vi "FT10xx系列_T1_sample_1.0.3.vi"() -> ()   [LabVIEW 2017]
uses:
  National Instruments/LabVIEW 2017/user.lib/smncsftmt/smncsftmt.lvlib
panel:
  out "数值 2":i32
  in  "分辨率":T1(ring)
  in  "分辨":T2(ring)
  in  "停止按钮":bool
  out "START 计数率":u32
  in  "开始测试":bool
  out "CH8 计数率":u32
  out "CH7 计数率":u32
  out "CH6 计数率":u32
  out "CH5 计数率":u32
  out "CH4 计数率":u32
  out "CH3 计数率":u32
  out "CH2 计数率":u32
  out "CH1 计数率":u32
  in  "Delay 8":dbl min=-1000.0 max=1000.0 step=0.1 format="%.1fns"
  in  "Delay 7":dbl min=-1000.0 max=1000.0 step=0.1 format="%.1fns"
  in  "Delay 6":dbl min=-1000.0 max=1000.0 step=0.1 format="%.1fns"
  in  "Delay 5":dbl min=-1000.0 max=1000.0 step=0.1 format="%.1fns"
  in  "Delay 4":dbl min=-1000.0 max=1000.0 step=0.1 format="%.1fns"
  in  "Delay 3":dbl min=-1000.0 max=1000.0 step=0.1 format="%.1fns"
  in  "Delay2":dbl min=-1000.0 max=1000.0 step=0.1 format="%.1fns"
  in  "Delay":dbl min=-1000.0 max=1000.0 step=0.1 format="%.1fns"
  in  "单选按钮 2":T3(radio)
  in  "保存路径":path=path "D:/siminics"
  in  "最大计数":u64=65535 min=1 max=4294967295 step=1
  in  "总采集时长（s)":sgl=1.0 min=0.1 max=604080 step=0.1
  out "TDC Controller":u64[](graph)
  out "采集次数":u32
  out "峰值计数":u32
  out "error out":errorcluster caption="错误输出"
  out "峰值时间点(ps)":u32
  out "已连接？":bool
  # "FT10XX系列直方图(T1)"
  # "通道选择"
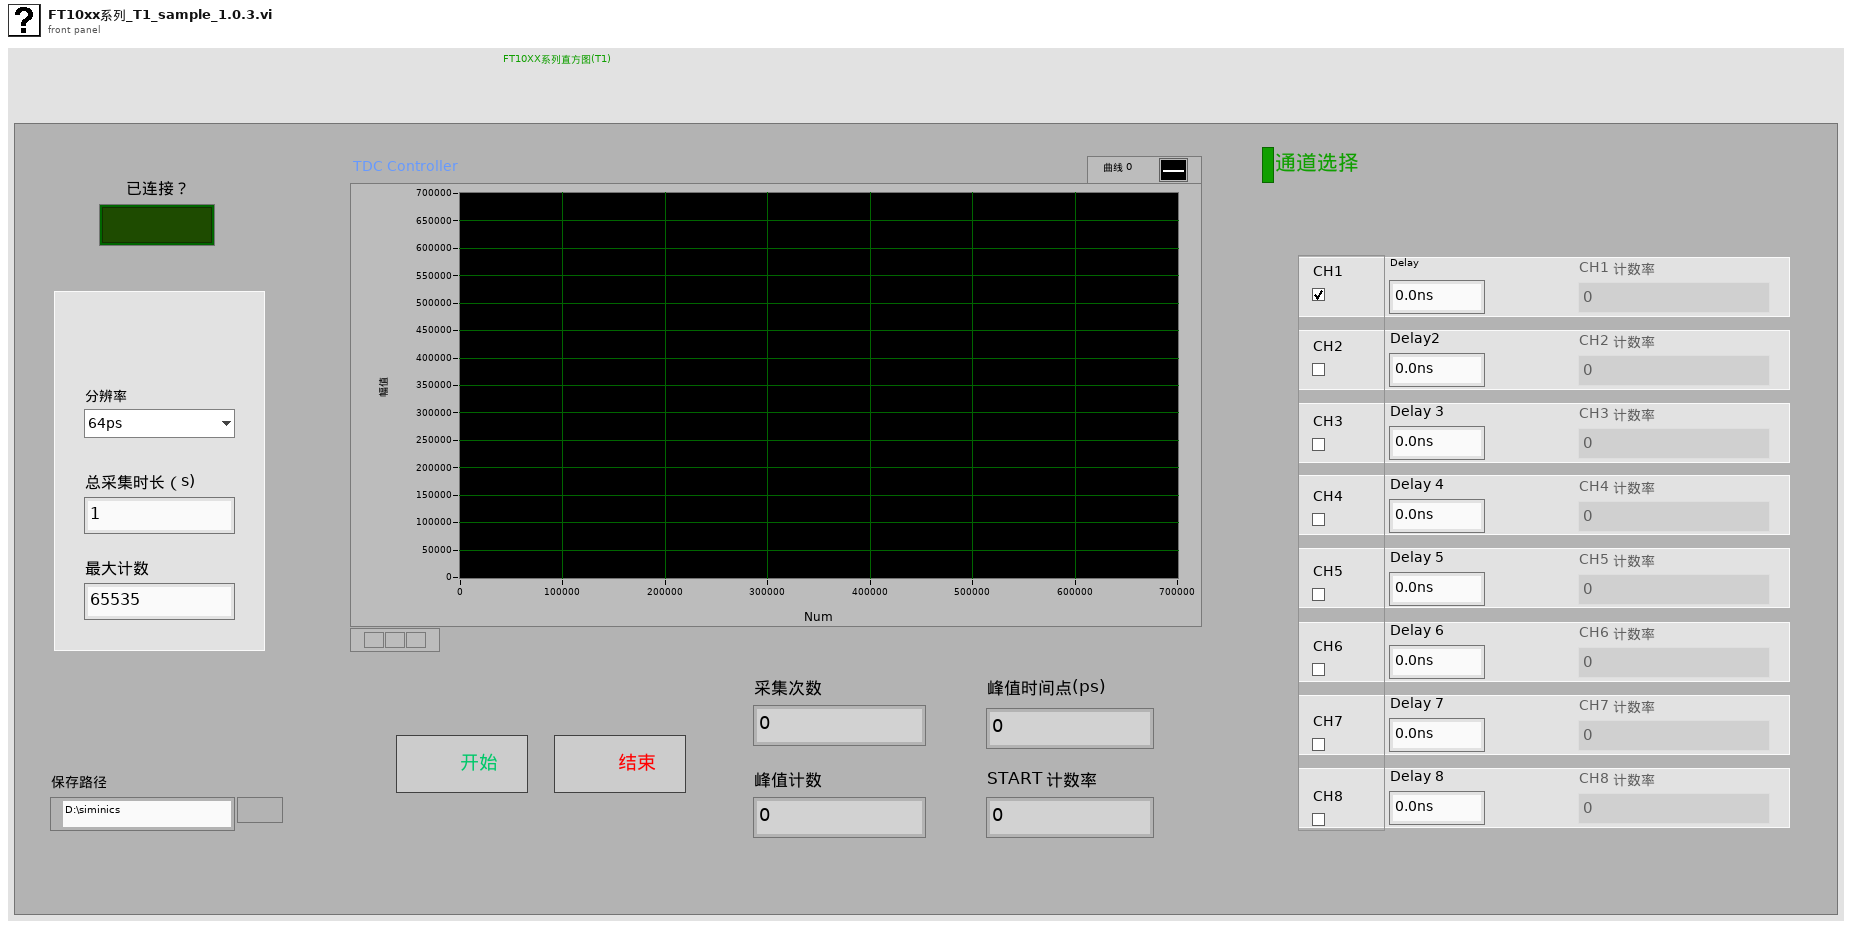
[diagram p1: front panel]
types:
  T1 = enum16{"64ps", "128ps", "256ps", "512ps", "1024ps", "2048ps", "4096ps", "8192ps", "16384ps", "32768ps", "65536ps", "131072ps", "262144ps", "524288ps", "1048576ps", "2097152ps", "4194304ps", "8388608ps", "16777216ps", "33554432ps"}
  T2 = enum16{"16ps", "32ps", "64ps", "128ps", "256ps", "512ps", "1024ps", "2048ps", "4096ps", "8192ps", "16384ps", "32768ps", "65536ps", "131072ps", "262144ps", "524288ps", "1048576ps", "2097152ps", "4194304ps", "8388608ps", "16777216ps", "33554432ps"}
  T3 = enum32{"CH1", "CH2", "CH3", "CH4", "CH5", "CH6", "CH7", "CH8"}
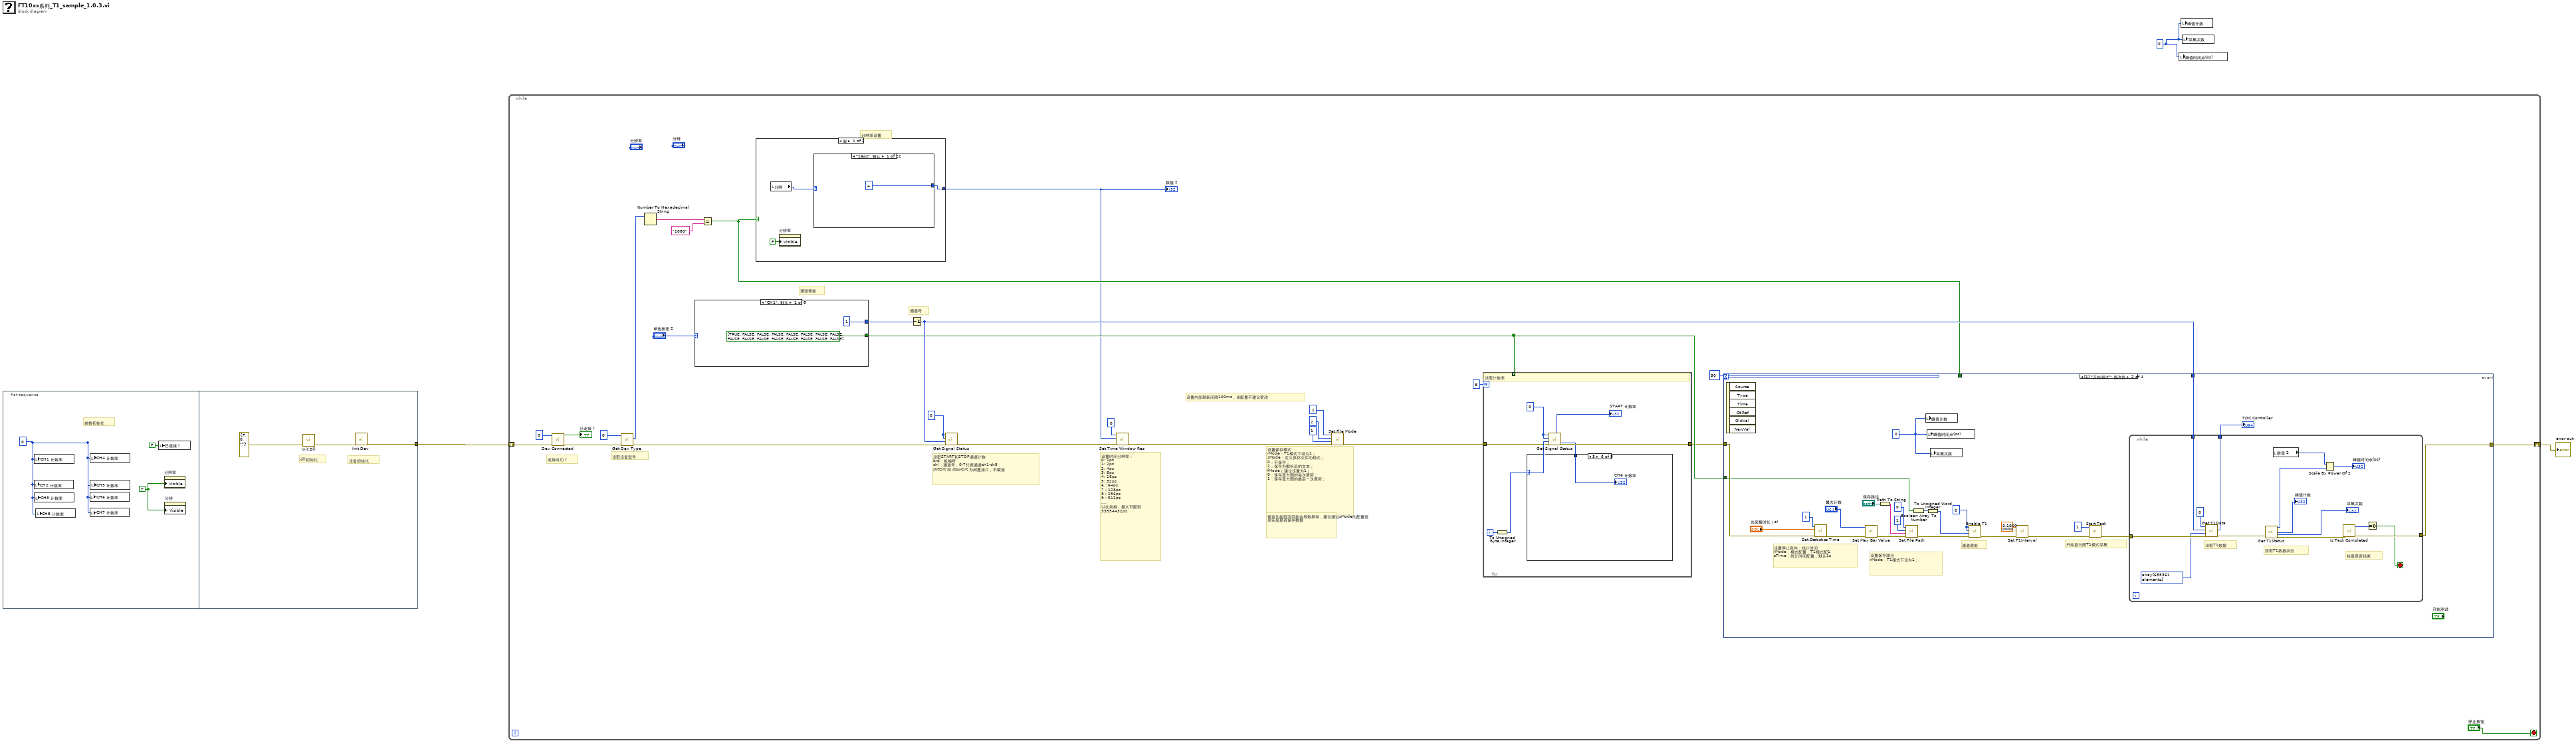
[diagram p0: block diagram]
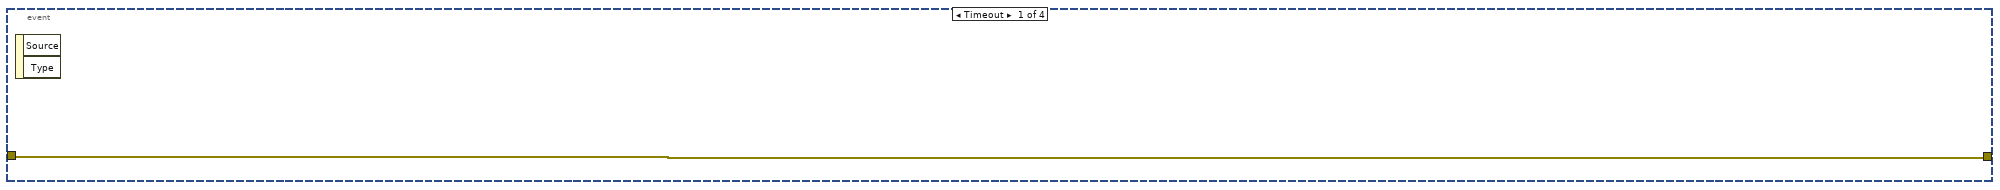
[diagram p2: hidden frame]
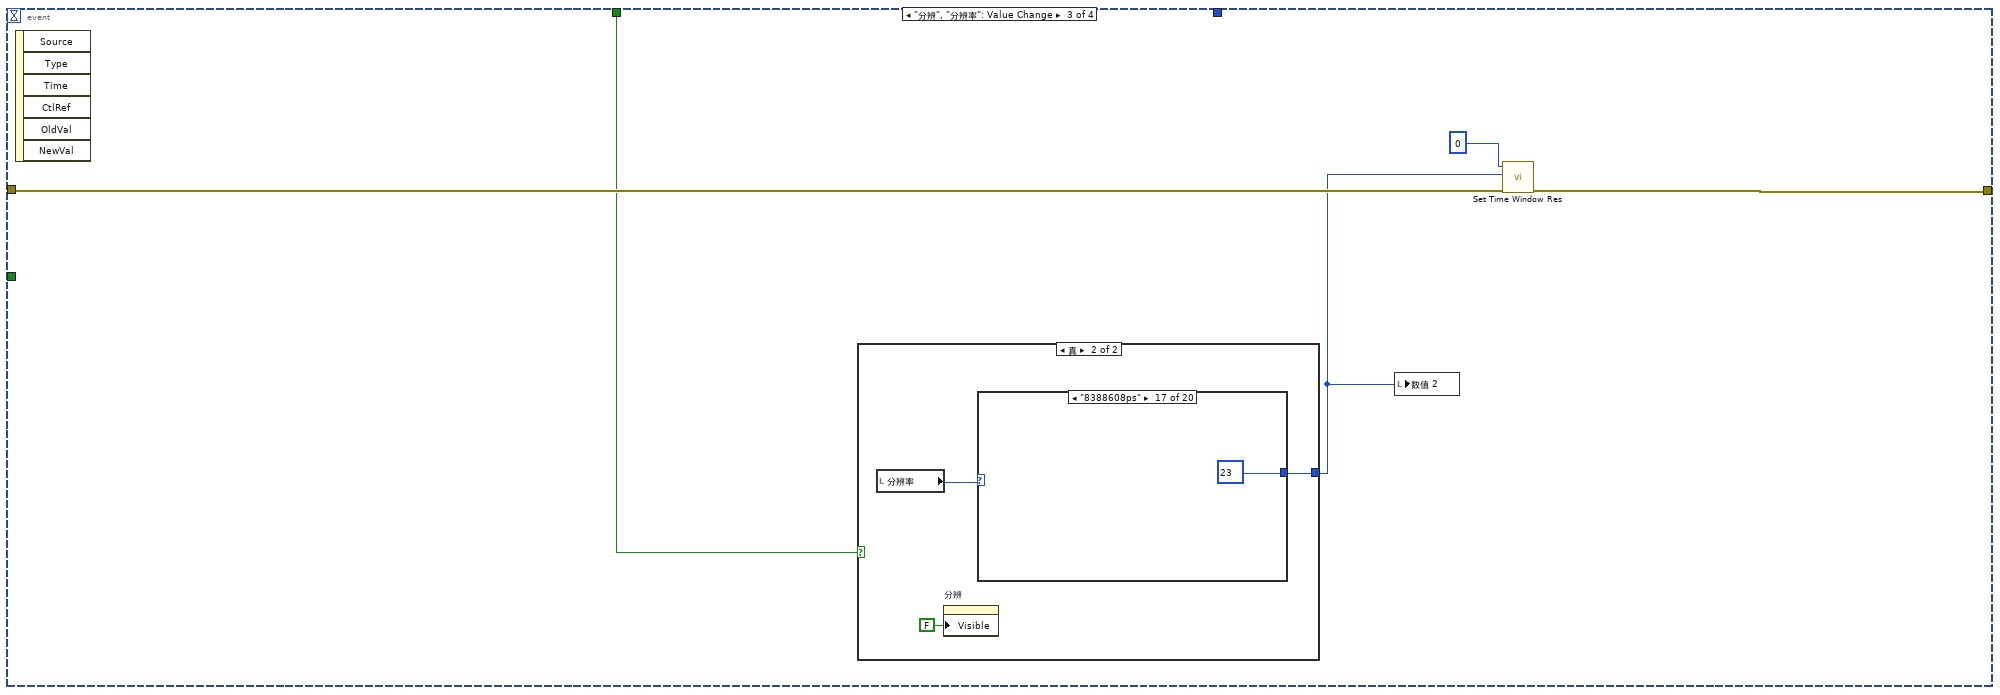
[diagram p3: hidden frame]
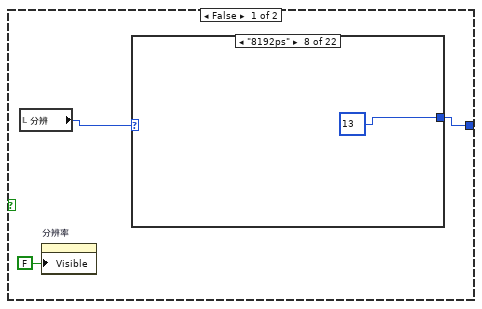
[diagram p4: hidden frame]
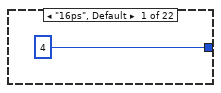
[diagram p5: hidden frame]
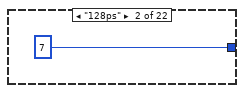
[diagram p6: hidden frame]
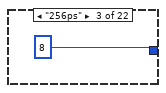
[diagram p7: hidden frame]
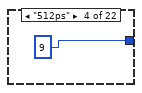
[diagram p8: hidden frame]
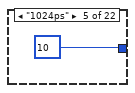
[diagram p9: hidden frame]
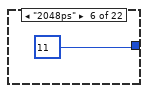
[diagram p10: hidden frame]
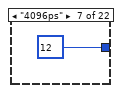
[diagram p11: hidden frame]
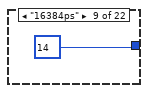
[diagram p12: hidden frame]
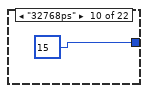
[diagram p13: hidden frame]
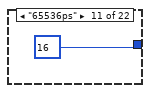
[diagram p14: hidden frame]
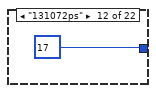
[diagram p15: hidden frame]
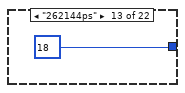
[diagram p16: hidden frame]
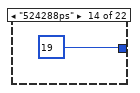
[diagram p17: hidden frame]
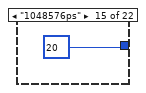
[diagram p18: hidden frame]
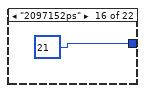
[diagram p19: hidden frame]
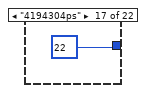
[diagram p20: hidden frame]
diagram:
  w1 = 0
  n1 = flat-sequence {
    tunnel: [w8] -> w3
    frame #0 {
      w4 = 0
      w5 = TRUE
      # "参数初始化"
      n2 = local write "CH2 计数率"(w4) -> ()
      n3 = local write "CH1 计数率"(w4) -> ()
      n4 = local write "CH3 计数率"(w4) -> ()
      n5 = local write "CH8 计数率"(w4) -> ()
      n6 = local write "CH6 计数率"(w4) -> ()
      n7 = local write "CH7 计数率"(w4) -> ()
      n8 = local write "CH4 计数率"(w4) -> ()
      n9 = local write "CH5 计数率"(w4) -> ()
      n10 = local write "已连接？"(FALSE ("已连接？")) -> ()
      n11 = property on="分辨率" class="Enum (严格)"("Visible"=w5) -> ()  [unwired: 2 in, 2 out]
      n12 = property on="分辨" class="Enum (严格)"("Visible"=w5) -> ()  [unwired: 2 in, 2 out]
    }
    frame #1 {
      # "设备初始化"
      # "dll初始化"
      n13 = call "Init Dll.vi"("error in (no error)"=errorcluster {"status"=FALSE, "code"=0, "source"=""}) -> ("error out"=w9:errorcluster)  [unwired: 9 in, 1 out]
      n14 = call "Init Dev.vi"("error in (no error)"=w9) -> ("error out"=w8:errorcluster)  [unwired: 9 in, 1 out]
    }
  }
  n15 = while {
    shift-right: [w28] -> w2
    shift-left: w3 -> [w16]
    stop <- "停止按钮" stop-if-true
    w33 = 0 ("brd")
    # "连接成功？"
    # "分辨率设置"
    # "读取设备型号"
    # "设置时间分辨率：\n0: 1ps\n1: 2ps\n2: 4ps\n3: 8ps\n4: 16ps\n5: 32ps\n6 : 64ps\n7 : 128ps\n8 : 256ps\n9 : 512ps\n....\n以此类推，最大可配到\n33554432ps"
    # "设置内部刷新间隔100ms，该配置不建议更改"
    # "通道号"
    # "通道使能"
    # "保存功能取消可能会导致异常，建议通过sMode的配置值来实现是否保存数据"
    # "设置保存模式\nrMode：T1模式下设为1；\nsMode：定义保存文件的格式；\n0：不保存；\n2：保存为解析后的文本；\nfMode（建议设置为1）：\n0：保存直方图的每次更新；\n1：保存直方图的最后一次更新；"
    # "读取START和STOP通道计数\nbrd：板编号\nchl：通道号，0-7代表通道ch1-ch8；\nstrtCnt 和 stopCnt 为闲置接口，不赋值"
    n16 = call "Dev Connected.vi"("error in (no error)"=w16, "nDevId"=0 ("devId")) -> ("error out"=w15:errorcluster, "function return"=→"已连接？":bool)  [unwired: 8 in]
    n17 = call "Get Dev Type.vi"("error in (no error)"=w15, "nDevId"=0 ("devId")) -> ("error out"=w26:errorcluster, "ptrType out"=w12:u32)  [unwired: 7 in, 1 out]
    n18 = Number To Hexadecimal String(2:w12) -> (0:w11:string)  [unwired: 1 in]
    n19 = case shown="\"CH1\", 默认" "单选按钮 2" {
      tunnel: [bool[] [TRUE, FALSE, FALSE, FALSE, FALSE, FALSE, FALSE, FALSE, FALSE, FALSE, FALSE, FALSE, FALSE, FALSE, FALSE, FALSE] bool[] [FALSE, TRUE, FALSE, FALSE, FALSE, FALSE, FALSE, FALSE, FALSE, FALSE, FALSE, FALSE, FALSE, FALSE, FALSE, FALSE] bool[] [FALSE, FALSE, TRUE, FALSE, FALSE, FALSE, FALSE, FALSE, FALSE, FALSE, FALSE, FALSE, FALSE, FALSE, FALSE, FALSE] bool[] [FALSE, FALSE, FALSE, TRUE, FALSE, FALSE, FALSE, FALSE, FALSE, FALSE, FALSE, FALSE, FALSE, FALSE, FALSE, FALSE] bool[] [FALSE, FALSE, FALSE, FALSE, TRUE, FALSE, FALSE, FALSE, FALSE, FALSE, FALSE, FALSE, FALSE, FALSE, FALSE, FALSE] bool[] [FALSE, FALSE, FALSE, FALSE, FALSE, TRUE, FALSE, FALSE, FALSE, FALSE, FALSE, FALSE, FALSE, FALSE, FALSE, FALSE] bool[] [FALSE, FALSE, FALSE, FALSE, FALSE, FALSE, TRUE, FALSE, FALSE, FALSE, FALSE, FALSE, FALSE, FALSE, FALSE, FALSE] bool[] [FALSE, FALSE, FALSE, FALSE, FALSE, FALSE, FALSE, TRUE, FALSE, FALSE, FALSE, FALSE, FALSE, FALSE, FALSE, FALSE]] -> w25
      tunnel: [1 2 3 4 5 6 7 8] -> w31
      frame "CH1", Default {
      }
      frame "CH2" {
      }
      frame "CH3" {
      }
      frame "CH4" {
      }
      frame "CH5" {
      }
      frame "CH6" {
      }
      frame "CH7" {
      }
      frame "CH8" {
      }
    }
    n20 = Equal?(x=w11, y="1080") -> (x = y?=w24:bool)
    n21 = case shown="假" w24 {
      tunnel: [w148 w173] -> w22
      frame False {
        n22 = local read "分辨"() -> (w149:T2)
        n23 = property on="分辨率" class="Enum (严格)"("Visible"=FALSE ("可见")) -> ()  [unwired: 2 in, 2 out]
        n24 = case shown="\"16ps\", 默认" w149 {
          tunnel: [4 7 8 9 10 11 12 13 14 15 16 17 18 19 20 21 22 23 24 25 6 5] -> w148
          frame "16ps", Default {
          }
          frame "128ps" {
          }
          frame "256ps" {
          }
          frame "512ps" {
          }
          frame "1024ps" {
          }
          frame "2048ps" {
          }
          frame "4096ps" {
          }
          frame "8192ps" {
          }
          frame "16384ps" {
          }
          frame "32768ps" {
          }
          frame "65536ps" {
          }
          frame "131072ps" {
          }
          frame "262144ps" {
          }
          frame "524288ps" {
          }
          frame "1048576ps" {
          }
          frame "2097152ps" {
          }
          frame "4194304ps" {
          }
          frame "8388608ps" {
          }
          frame "16777216ps" {
          }
          frame "33554432ps" {
          }
          frame "64ps" {
          }
          frame "32ps" {
          }
        }
      }
      frame True {
        n25 = local read "分辨率"() -> (w174:T1)
        n26 = property on="分辨" class="Enum (严格)"("Visible"=FALSE ("可见")) -> ()  [unwired: 2 in, 2 out]
        n27 = case shown="\"1024ps\"" w174 {
          tunnel: [7 8 9 10 11 12 13 14 15 16 17 18 19 20 21 22 23 24 25 6] -> w173
          frame "128ps" {
          }
          frame "256ps" {
          }
          frame "512ps" {
          }
          frame "1024ps" {
          }
          frame "2048ps" {
          }
          frame "4096ps" {
          }
          frame "8192ps" {
          }
          frame "16384ps" {
          }
          frame "32768ps" {
          }
          frame "65536ps" {
          }
          frame "131072ps" {
          }
          frame "262144ps" {
          }
          frame "524288ps" {
          }
          frame "1048576ps" {
          }
          frame "2097152ps" {
          }
          frame "4194304ps" {
          }
          frame "8388608ps" {
          }
          frame "16777216ps" {
          }
          frame "33554432ps" {
          }
          frame "64ps" {
          }
        }
      }
    }
    "数值 2" <- w22
    n28 = Decrement(x=w31) -> (x-1=w30:i32)
    n29 = call "Get Signal Status.vi"("error in (no error)"=w26, "nChannel"=w30, "nBoard"=w33, "nDevId"=w33) -> ("error out"=w37:errorcluster)  [unwired: 4 in, 3 out]
    n30 = call "Set Time Window Res.vi"("error in (no error)"=w37, "nWinRes"=w22, "nDevId"=0) -> ("error out"=w23:errorcluster)  [unwired: 7 in, 1 out]
    n31 = call "Set File Mode.vi"("error in (no error)"=w23, "nFilterMode"=1 ("fMode"), "nSaveMode"=2 ("sMode"), "nRunMode"=1 ("rMode")) -> ("error out"=w29:errorcluster)  [unwired: 6 in, 1 out]
    n32 = for {
      N: 8 -> [_]
      tunnel: w25 -> [_] mode=indexing
      tunnel: w29 -> [w216]
      tunnel: [w215] -> w19
      i -> [w218]
      w213 = 0
      # "读取计数率"
      n33 = To Unsigned Byte Integer(number=w218) -> (unsigned 8bit integer=w217:u8)
      n34 = call "Get Signal Status.vi"("error in (no error)"=w216, "nChannel"=w217, "nBoard"=w213, "nDevId"=w213) -> ("error out"=w215:errorcluster, "ptrStopCount out"=w214:u32, "ptrStartCount out"=→"START 计数率":u32)  [unwired: 4 in, 1 out]
      n35 = case shown="5" w217 {
        tunnel: w214 -> [w219 w220 w221 w222 w223 w224 w225 w226]
        frame 0, Default {
          "CH1 计数率" <- w219
        }
        frame 1 {
          "CH2 计数率" <- w220
        }
        frame 2 {
          "CH3 计数率" <- w221
        }
        frame 3 {
          "CH4 计数率" <- w222
        }
        frame 4 {
          "CH5 计数率" <- w223
        }
        frame 5 {
          "CH6 计数率" <- w224
        }
        frame 6 {
          "CH7 计数率" <- w225
        }
        frame 7 {
          "CH8 计数率" <- w226
        }
      }
    }
    n36 = event shown="[1] \"开始测试\": 值改变" {
      selector: _ -> [_ _ _ _]
      dyn-events: _ -> [_ _ _ _]
      timeout: 50 -> [_ _ _ _]
      tunnel: w30 -> [_ w59 _ _]
      tunnel: w19 -> [w38 w48 w81 w132]
      tunnel: [w38 w58 w80 w131] -> w28
      tunnel: w25 -> [_ w42 _ _]
      tunnel: w24 -> [_ _ w79 _]
      event Timeout {
        n37 = event-data() -> ()  [unwired: 1 in, 2 out]
      }
      event "开始测试": Value Change {
        w51 = 0
        w57 = 0 ("brd")
        # "设置停止条件：统计时间\nrMode：模式配置，T1模式配1\nsTime：统计时间配置，默认1s"
        # "设置保存路径\nrMode：T1模式下设为1；"
        # "通道使能"
        # "开始直方图T1模式采集"
        n38 = event-data() -> ()  [unwired: 1 in, 6 out]
        n39 = call "Set Statistics Time.vi"("error in (no error)"=w48, "Times"="总采集时长（s)", "nRunMode"=1) -> ("error out"=w50:errorcluster)  [unwired: 7 in, 1 out]
        n40 = call "Set Max Bar Value.vi"("error in (no error)"=w50, "uValue64"="最大计数") -> ("error out"=w47:errorcluster)  [unwired: 8 in, 1 out]
        n41 = Path To String(path="保存路径") -> (string=w56:string)
        n42 = call "Set File Path.vi"("error in (no error)"=w47, "strFilePath"=w56, "nRunMode"=1 ("rMode"), "nDevId"=0) -> ("error out"=w52:errorcluster)  [unwired: 6 in, 1 out]
        n43 = Boolean Array To Number(Boolean array=w42) -> (number=w44:u32)
        n44 = local write "峰值计数"(w51) -> ()
        n45 = local write "峰值时间点(ps)"(w51) -> ()
        n46 = To Unsigned Word Integer(number=w44) -> (unsigned 16bit integer=w43:u16)
        n47 = local write "采集次数"(w51) -> ()
        n48 = call "Enable T1.vi"("error in (no error)"=w52, "uMask16"=w43, "nBoard"=w57, "nDevId"=w57) -> ("error out"=w41:errorcluster)  [unwired: 6 in, 1 out]
        n49 = call "Set T1Interval.vi"("error in (no error)"=w41, "fIntvl"=sgl 0.1) -> ("error out"=w40:errorcluster)  [unwired: 8 in, 1 out]
        n50 = call "Start Task.vi"("error in (no error)"=w40, "nRunMode"=1 ("rMode")) -> ("error out"=w61:errorcluster)  [unwired: 8 in, 1 out]
        n51 = while {
          tunnel: w61 -> [w73]
          tunnel: [w77] -> w58
          tunnel: [w65] -> w62
          tunnel: w59 -> [w70]
          stop <- w66 stop-if-true
          # "读取T1数据"
          # "检查是否结束"
          # "获取T1数据状态"
          n52 = call "Get T1Data.vi"("error in (no error)"=w73, "data"=u64[] array[655361 elements], "nChannel"=w70, "nBoard"=0 ("brd")) -> ("error out"=w74:errorcluster, "data 2"=w65:u64[])  [unwired: 5 in, 1 out]
          n53 = call "Get T1Status.vi"("error in (no error)"=w74) -> ("uXMax out"=w72:u32, "uYMax 2"=→"峰值计数":u64, "uCount out"=→"采集次数":u32, "error out"=w69:errorcluster)  [unwired: 8 in, 3 out]
          n54 = local read "数值 2"() -> (w68:i32)
          n55 = Scale By Power Of 2(n=w68, x=w72) -> (x*2^n=→"峰值时间点(ps)":u32)
          n56 = call "Is Task Completed.vi"("error in (no error)"=w69) -> ("error out"=w77:errorcluster, "function return"=w67:i32)  [unwired: 9 in]
          n57 = Equal To 0?(x=w67) -> (x = 0?=w66:bool)
        }
        "TDC Controller" <- w62
      }
      event "分辨", "分辨率": Value Change {
        n58 = event-data() -> ()  [unwired: 1 in, 6 out]
        n59 = case shown="真" w79 {
          tunnel: [w83 w108] -> w78
          frame False {
            n60 = local read "分辨"() -> (w84:T2)
            n61 = property on="分辨率" class="Enum (严格)"("Visible"=FALSE ("可见")) -> ()  [unwired: 2 in, 2 out]
            n62 = case shown="\"8192ps\"" w84 {
              tunnel: [4 7 8 9 10 11 12 13 14 15 16 17 18 19 20 21 22 23 24 25 6 5] -> w83
              frame "16ps", Default {
              }
              frame "128ps" {
              }
              frame "256ps" {
              }
              frame "512ps" {
              }
              frame "1024ps" {
              }
              frame "2048ps" {
              }
              frame "4096ps" {
              }
              frame "8192ps" {
              }
              frame "16384ps" {
              }
              frame "32768ps" {
              }
              frame "65536ps" {
              }
              frame "131072ps" {
              }
              frame "262144ps" {
              }
              frame "524288ps" {
              }
              frame "1048576ps" {
              }
              frame "2097152ps" {
              }
              frame "4194304ps" {
              }
              frame "8388608ps" {
              }
              frame "16777216ps" {
              }
              frame "33554432ps" {
              }
              frame "64ps" {
              }
              frame "32ps" {
              }
            }
          }
          frame True {
            n63 = local read "分辨率"() -> (w109:T1)
            n64 = property on="分辨" class="Enum (严格)"("Visible"=FALSE ("可见")) -> ()  [unwired: 2 in, 2 out]
            n65 = case shown="\"8388608ps\"" w109 {
              tunnel: [7 8 9 10 11 12 13 14 15 16 17 18 19 20 21 22 23 24 25 6] -> w108
              frame "128ps" {
              }
              frame "256ps" {
              }
              frame "512ps" {
              }
              frame "1024ps" {
              }
              frame "2048ps" {
              }
              frame "4096ps" {
              }
              frame "8192ps" {
              }
              frame "16384ps" {
              }
              frame "32768ps" {
              }
              frame "65536ps" {
              }
              frame "131072ps" {
              }
              frame "262144ps" {
              }
              frame "524288ps" {
              }
              frame "1048576ps" {
              }
              frame "2097152ps" {
              }
              frame "4194304ps" {
              }
              frame "8388608ps" {
              }
              frame "16777216ps" {
              }
              frame "33554432ps" {
              }
              frame "64ps" {
              }
            }
          }
        }
        n66 = local write "数值 2"(w78) -> ()
        n67 = call "Set Time Window Res.vi"("error in (no error)"=w81, "nWinRes"=w78, "nDevId"=0 ("devId")) -> ("error out"=w80:errorcluster)  [unwired: 7 in, 1 out]
      }
      event "Delay", "Delay2", "Delay 3", "Delay 4", "Delay 5", "Delay 6", "Delay 7", "Delay 8": Value Change {
        # "Delay延时"
        n68 = event-data() -> ()  [unwired: 1 in, 6 out]
        n69 = local read "Delay"() -> (w140:dbl)
        n70 = local read "Delay2"() -> (w139:dbl)
        n71 = local read "Delay 3"() -> (w138:dbl)
        n72 = local read "Delay 4"() -> (w137:dbl)
        n73 = local read "Delay 5"() -> (w136:dbl)
        n74 = local read "Delay 6"() -> (w135:dbl)
        n75 = local read "Delay 7"() -> (w134:dbl)
        n76 = local read "Delay 8"() -> (w133:dbl)
        n77 = Build Array(w140, w139, w138, w137, w136, w135, w134, w133) -> (w141:dbl[])
        n78 = for {
          shift-right: [w145] -> w131
          shift-left: w132 -> [w146]
          tunnel: w141 -> [w144] mode=indexing
          i -> [w143]
          w147 = 0
          n79 = To Unsigned Byte Integer(number=w143) -> (unsigned 8bit integer=w142:u8)
          n80 = call "Set Stop Delay.vi"("fDelay"=w144, "error in (no error)"=w146, "nChannel"=w142, "nBoard"=w147, "nDevId"=w147) -> ("error out"=w145:errorcluster)  [unwired: 5 in, 1 out]
        }
      }
    }
  }
  "error out" <- w2
  n81 = local write "峰值时间点(ps)"(w1) -> ()
  n82 = local write "峰值计数"(w1) -> ()
  n83 = local write "采集次数"(w1) -> ()
